vi "SubscribeAnyUpdated Start Stream.vi"(8 "timeout":i32=-1, 9 "gRPCid":T2, 10 "Event Registration Refnum in":refnum<event-registration>) -> (0 "error out":errorcluster, 2 "Event Registration Refnum out":refnum<event-registration>, 3 "Stream Data out":T1={"gRPCid"=0, "Active"=FALSE, "timeout"=-1})   [LabVIEW 2020]
doc: "Starting process for broadcasts:\n- build <b>Stream Data</b> cluster with provided parameters (Active is always set to true). If no timeout is provided the default value -1 is set.\n- Register <b>Broadcast Events</b> of DQMH module."
uses:
  <vilib>/gRPC/LabVIEW gRPC Library/Server API/typeDefs/gRPCId Cluster.ctl
  <vilib>/gRPC/LabVIEW gRPC Library/Shared/grpcId.ctl
  thermal-chamber-controller_server/RPC Service/ThermalChamberController/typeDefs/Server Internal Message.ctl
  Stream Data--cluster.ctl
  Program Files (x86)/National Instruments/LabVIEW 2020/examples/DQMH Consortium/DQMH Fundamentals - Thermal Chamber/Libraries/Thermal Chamber Controller_DQMH/Thermal Chamber Controller_DQMH.lvlib
  <vilib>/gRPC/LabVIEW gRPC Library/grpc-lvsupport-release.lvlib
  thermal-chamber-controller_server/RPC Service/ThermalChamberController/ThermalChamberController.lvclass
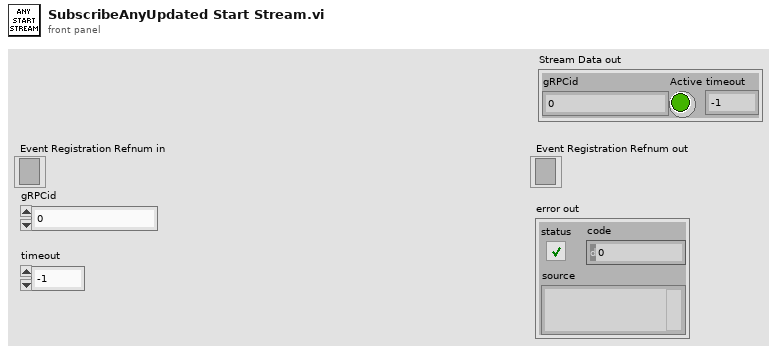
[diagram p1: front panel]
types:
  T1 = typedef "Stream Data--cluster.ctl" = cluster{"gRPCid":T2, "Active":bool, "timeout":i32}
  T2 = typedef "grpc-lvsupport-release.lvlib/grpcId.ctl" = u64
  T3 = typedef "Thermal Chamber Controller_DQMH.lvlib/Broadcast Events--cluster.ctl" = cluster{"Module Did Init":refnum<user-event>, "Status Updated":refnum<user-event>, "Error Reported":refnum<user-event>, "Module Did Stop":refnum<user-event>, "Update Module Execution Status":refnum<user-event>, "Chamber Status Updated":refnum<user-event>, "Set Point Updated":refnum<user-event>, "Ramp Rate Updated":refnum<user-event>, "Heater State Updated":refnum<user-event>}
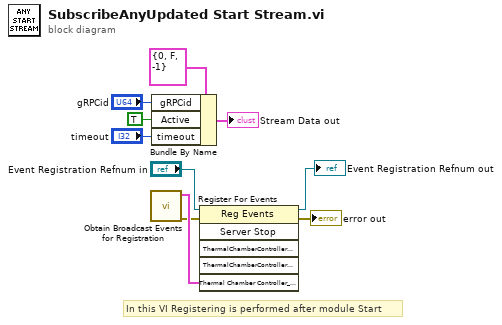
[diagram p0: block diagram]
diagram:
  # "In this VI Registering is performed after module Start"
  n1 = call "Obtain Broadcast Events for Registration.vi"() -> ("error out"=w8:errorcluster, "Thermal Chamber Controller_DQMH Broadcast Events"=w9:T3)  [unwired: 9 in, 1 out]
  n2 = Bundle By Name(cluster=T1 {"gRPCid"=0, "Active"=FALSE, "timeout"=-1} ("Stream Data in"), "gRPCid"="gRPCid", "Active"=TRUE, "timeout"="timeout") -> (→"Stream Data out":T1)
  n3 = register-events(reference="Event Registration Refnum in", error in=w8, w9) -> (reference out=→"Event Registration Refnum out":refnum<event-registration>, error out=→"error out":errorcluster)  [unwired: 3 in]
